vi "Get Matrix of U32.vi"(8 "error in (no error)":errorcluster, 10 "Name":string, 11 "json class in":refnum<class "json class.lvclass">) -> (0 "error out":errorcluster, 2 "Array":u32[][](array[numeric]), 3 "json class out":refnum<class "json class.lvclass">)   [LabVIEW 2021, in "Config Library.lvlib" / "json class.lvclass"]
uses:
  json class.lvclass
  json class.lvclass/json class.ctl
  <vilib>/addons/JSON API/JSON Value/JSON Value.lvclass
  <vilib>/addons/JSON API/JSON Scalar/JSON Scalar.lvclass
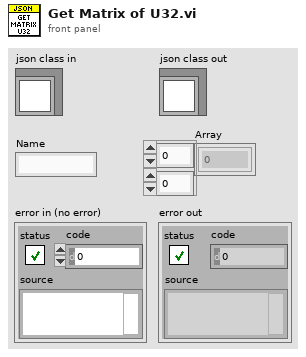
[diagram p1: front panel]
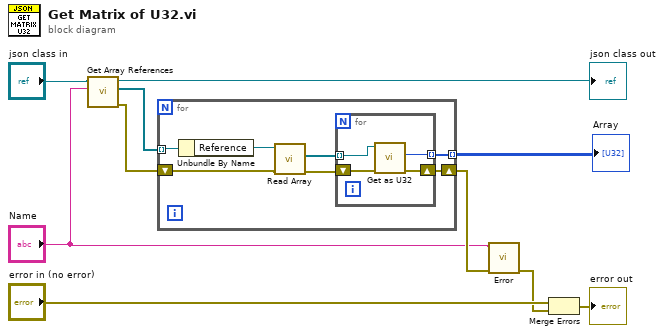
[diagram p0: block diagram]
diagram:
  n1 = call "Get Array References.vi"("Name"="Name", "json class in"="json class in") -> ("error out"=w5:errorcluster, "Array json class"=w6:refnum<class "json class.lvclass">[], "json class out"=→"json class out":refnum<class "json class.lvclass">)  [unwired: 7 in]
  n2 = for {
    tunnel: w6 -> [w17] mode=indexing
    tunnel: [w15] -> w7 mode=indexing
    shift-right: [w16] -> w4
    shift-left: w5 -> [w12]
    n3 = Unbundle By Name(w17) -> ("Reference"=w14:refnum<class "JSON Value.lvclass">)
    n4 = call-dynamic "Read Array.vi"("error in (no error)"=w12, "JSON Value In"=w14) -> ("error out"=w11:errorcluster, "Array"=w13:refnum<class "JSON Value.lvclass">[])  [unwired: 7 in, 1 out]
    n5 = for {
      tunnel: [w19] -> w15 mode=indexing
      shift-right: [w20] -> w16
      shift-left: w11 -> [w21]
      tunnel: w13 -> [w18] mode=indexing
      n6 = call <vilib>:"Get as U32.vi"("error in (no error)"=w21, "JSON Scalar in"=w18) -> ("error out"=w20:errorcluster, "Number"=w19:u32)  [unwired: 7 in, 1 out]
    }
  }
  "Array" <- w7
  n7 = call "Error.vi"("error in (no error)"=w4, "Name"="Name") -> ("error out"=w2:errorcluster)  [unwired: 9 in]
  n8 = Merge Errors("error in (no error)", w2) -> (→"error out":errorcluster)
